vi "set Trigger Level.vi"(8 "error in (no error)":errorcluster, 10 "Trigger Level (dBm)":dbl, 11 "Keysight 9020A in":refnum<class "Keysight 9020A.lvclass">) -> (0 "error out":errorcluster, 3 "Keysight 9020A out":refnum<class "Keysight 9020A.lvclass">)   [LabVIEW 2023, in "Spectrum Analyzer.lvlib" / "Keysight 9020A.lvclass"]
uses:
  Keysight 9020A.lvclass
  Keysight 9020A.lvclass/Keysight 9020A.ctl
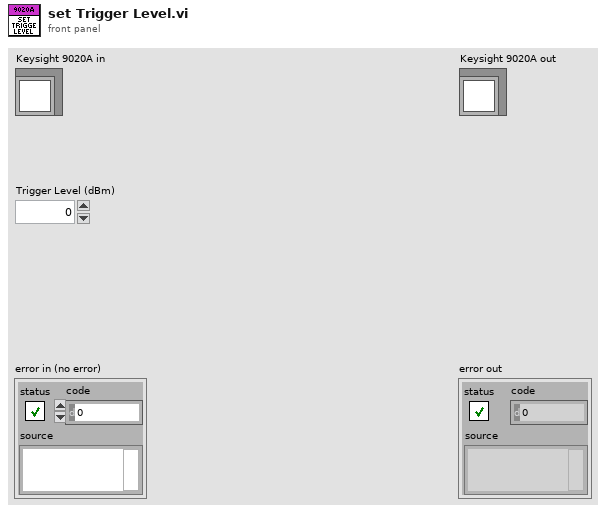
[diagram p1: front panel]
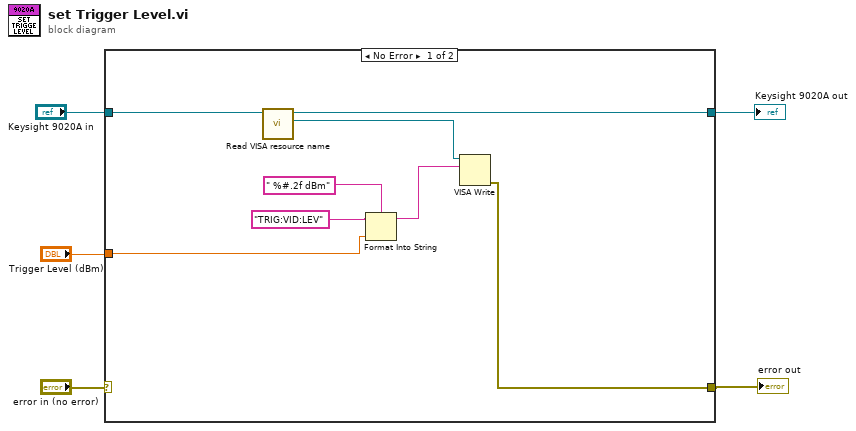
[diagram p0: block diagram]
diagram:
  n1 = case shown="No Error" "error in (no error)" {
    selector: "error in (no error)" -> [_ w14]
    tunnel: "Keysight 9020A in" -> [w9 w15]
    tunnel: [w13 w15] -> w4
    tunnel: [w6 w14] -> w2
    tunnel: "Trigger Level (dBm)" -> [w7 _]
    frame No Error {
      n2 = call "Read VISA resource name.vi"("Keysight 9020A in"=w9) -> ("VISA resource name"=w10:refnum<visa-resource-name>, "Keysight 9020A out"=w13:refnum<class "Keysight 9020A.lvclass">)  [unwired: 8 in, 1 out]
      n3 = Format Into String(format string=" %#.2f dBm", initial string="TRIG:VID:LEV", w7) -> (resulting string=w12:string)  [unwired: 1 in, 1 out]
      n4 = VISA Write(VISA resource name=w10, write buffer=w12) -> (error out=w6:errorcluster)  [unwired: 1 in, 2 out]
    }
    frame Error {
    }
  }
  "error out" <- w2
  "Keysight 9020A out" <- w4
